vi "Config_Validate_Target.vi"(8 "error in (no error)":errorcluster={"status"=FALSE, "code"=0, "source"="\"\""}, 10 "deployed capabilities":string, 11 "Decoded config":string) -> (0 "error out":errorcluster={"status"=FALSE, "code"=0, "source"="\"\""}, 2 "status ok":bool, 3 "Diagnostics and validity flag":string)   [LabVIEW 2026]
doc: "INTENT: Enforce target-specific validation. LOGIC: Check IDs, units, bounds, cyclic depth, resources, plugin manifests, device capabilities and controller modes."
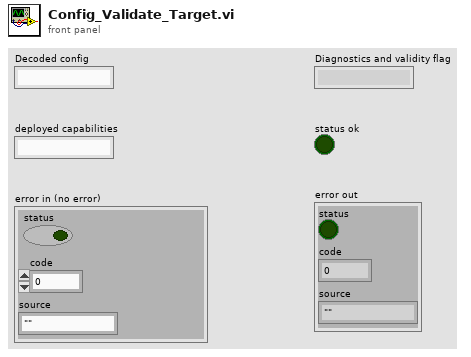
[diagram p1: front panel]
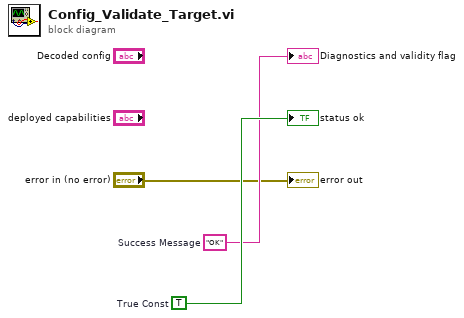
[diagram p0: block diagram]
diagram:
  w3 = TRUE  # True Const
  w2 = "OK"  # Success Message
  "Diagnostics and validity flag" <- w2
  "status ok" <- w3
  "error out" <- "error in (no error)"
